vi "Variable glob generale.vi"() -> ()   [LabVIEW 2022 SP3]
panel:
  out "MDP":string
  in  "Chemin fichier logbook :":path
  out "erreurs a enregistrer":string
  in  "Dossier prog":path
  in  "Chemin du fichier distant :":path
  out "Sous-dossier":string
  in  "Commentaire":string
  in  "Arret":bool
  in  "Gestion EUROTHERM en cours":bool
  in  "Profil EUROTHERM en cours":bool
  out "Visu donnees":i32[](array[numeric])
  in  "Dossier cuve distant":path
  in  "Visu en cours":bool
  out "Couleurs":u32[](array[colorbox])=[16754848, 16751217, 13132800, 16761130, 16773465, 9568042, 4390847, 40787, 1228799, 4358143, 9948, 5570815, 12587775, 16085503, 10420329, 16728690]
  out "Nom manip":string
  out "Date debut":timestamp
  in  "Chemin du fichier local :":path
  out "Entete fichier":string
  in  "Dossier sauvegarde":path
  in  "Lancement":bool caption="Arret"
  in  "Config OK":bool
  in  "Acqui tout":bool
  in  "Dossier cuve local":path
  out "Nom cuve":string
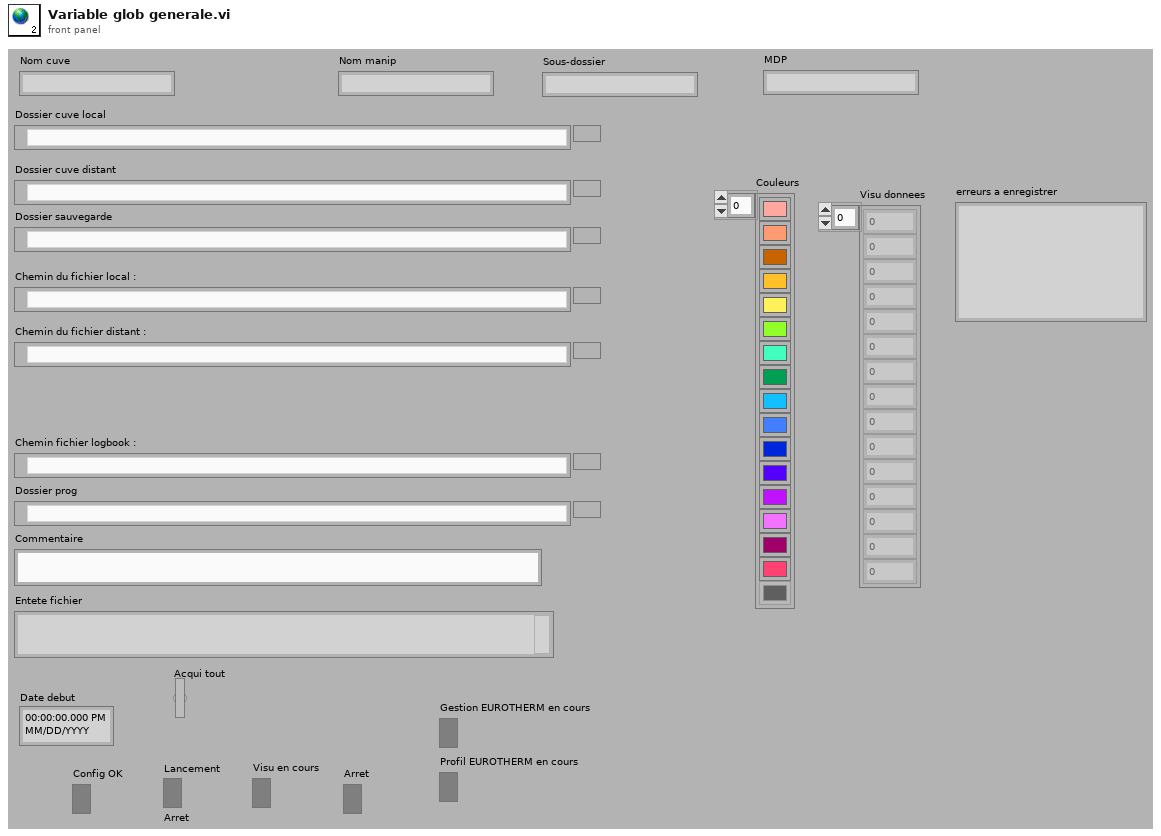
[diagram p1: front panel]
diagram:
